vi "RFH-verify-R140_conversion.vi"(5 "Conversion Folder":path, 7 "Excel File Folder":path, 8 "error in (no error)":errorcluster, 9 "Max Frequency (6G)":dbl=6000000000.0, 10 "Min Frequency  (0.3G)":dbl=300000000.0) -> (0 "error out":errorcluster, 2 "All Good?":bool)   [LabVIEW 2020, in "RFH-Reflection_File_Handler.lvlib"]
doc: "Verifies converted R140 files against their Excel source files, value by value and in the min and max frequency range. Returns whether all are good."
uses:
  RFH-Reflection_File_Handler.lvlib
  RFH-common_data_format_element.ctl
panel:
  out "Range Good?":bool
  out "Values Good?":bool
  out "All Files in Dir":path[](array[path])
  out "value 4":T1
  out "value 3":T1
  out "value 2":T1
  out "value":T1
  out "Array":bool[](array[boolean])
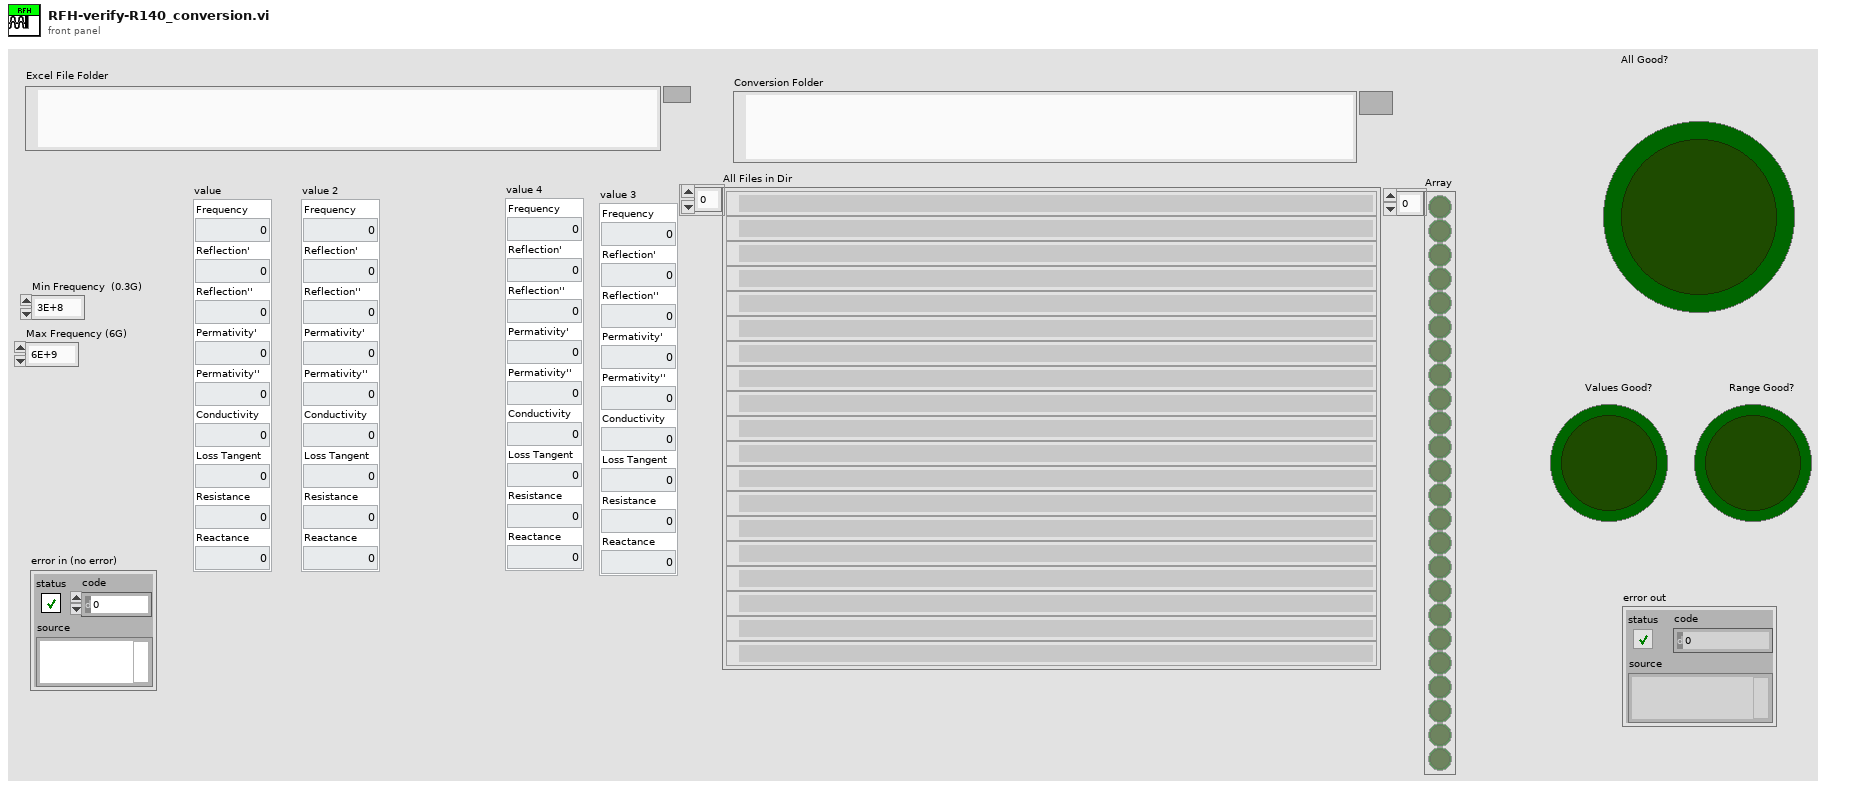
[diagram p1: front panel]
types:
  T1 = typedef "RFH-Reflection_File_Handler.lvlib/RFH-common_data_format_element.ctl" = cluster{"Frequency":dbl, "Reflection'":dbl, "Reflection''":dbl, "Permativity'":dbl, "Permativity''":dbl, "Conductivity":dbl, "Loss Tangent":dbl, "Resistance":dbl, "Reactance":dbl}
  T2 = typedef "RFH-Reflection_File_Handler.lvlib/RFH-common_data_format.ctl" = cluster{"Frequency":dbl[], "Reflection'":dbl[], "Reflection''":dbl[], "Permativity'":dbl[], "Permativity''":dbl[], "Conductivity":dbl[], "Loss Tangent":dbl[], "Resistance":dbl[], "Reactance":dbl[]}
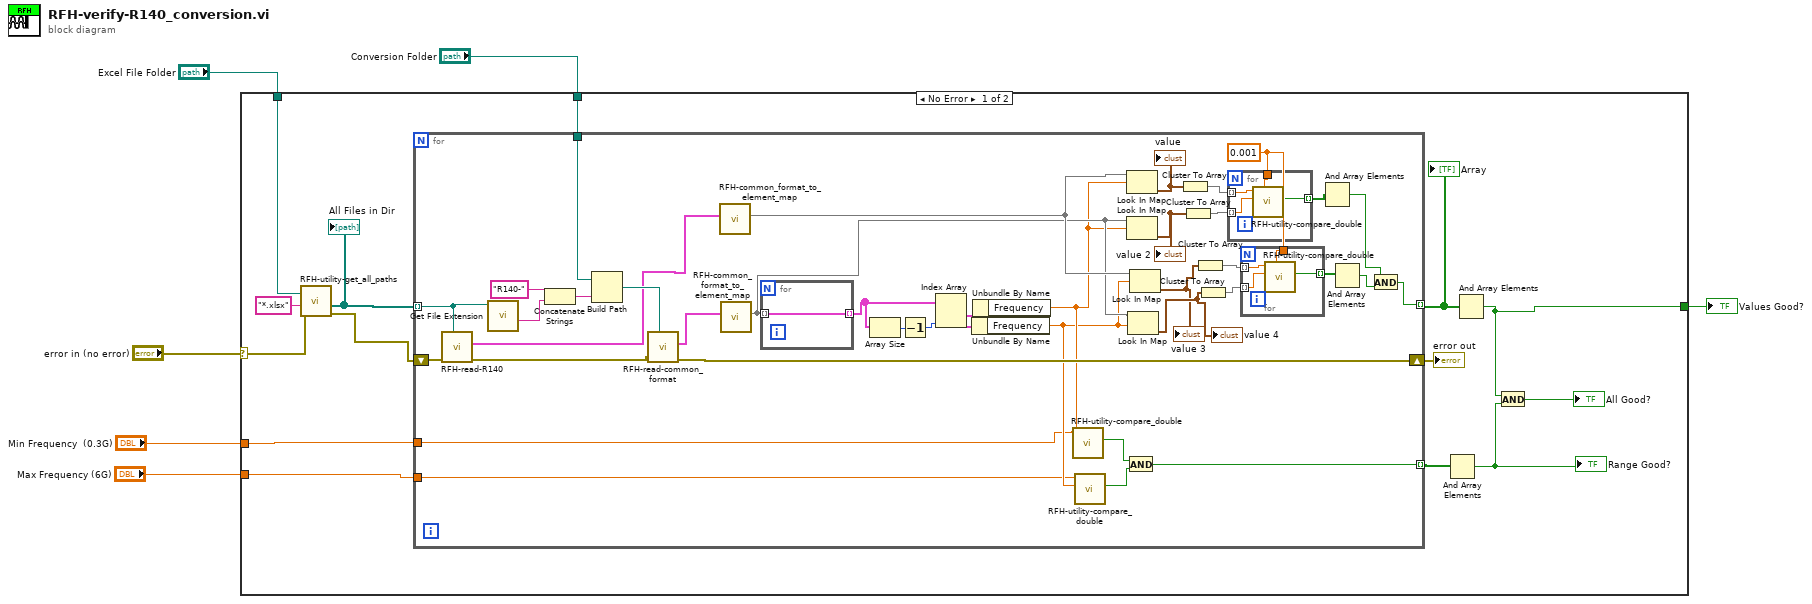
[diagram p0: block diagram]
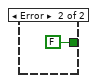
[diagram p2: hidden frame]
diagram:
  n1 = case shown="No Error" "error in (no error)" {
    selector: "error in (no error)" -> [w7 _]
    tunnel: "Excel File Folder" -> [w16 _]
    tunnel: "Conversion Folder" -> [w15 _]
    tunnel: "Min Frequency  (0.3G)" -> [w13 _]
    tunnel: "Max Frequency (6G)" -> [w12 _]
    tunnel: [w8 FALSE] -> w2
    frame No Error {
      n2 = call "RFH-utility-get_all_paths.vi"("Folder Path"=w16, "error in (no error)"=w7, "pattern"="*.xlsx") -> ("error out"=w19:errorcluster, "All Files in Dir"=w20:path[])  [unwired: 5 in, 2 out]
      "All Files in Dir" <- w20
      n3 = for {
        tunnel: w20 -> [w59] mode=indexing
        tunnel: w15 -> [w56]
        shift-right: [w51] -> w18
        shift-left: w19 -> [w54]
        tunnel: [w41] -> w14 mode=indexing
        tunnel: w13 -> [w23]
        tunnel: w12 -> [w22]
        tunnel: [w21] -> w10 mode=indexing
        w28 = 0.001 ("% tolerance (0.1)")
        n4 = call "RFH-read-R140.vi"("file path (dialog if empty)"=w59, "error in (no error)"=w54) -> ("error out"=w52:errorcluster, "Common Format"=w50:T2)  [unwired: 7 in, 1 out]
        n5 = call <vilib>:"Get File Extension.vi"("file"=w59) -> ("filename without extension"=w58:string)  [unwired: 6 in, 4 out]
        n6 = Concatenate Strings("R140-" ("string"), w58) -> (w57:string)
        n7 = Build Path(base path=w56, name or relative path=w57) -> (appended path=w53:path)
        n8 = call "RFH-read-common_format.vi"("file path (dialog if empty)"=w53, "error in"=w52) -> ("error out"=w51:errorcluster, "Common Format"=w49:T2)  [unwired: 8 in]
        n9 = call "RFH-common_format_to_element_map.vi"("Common Format"=w50) -> ("Element map"=w43:map{dbl, T1})  [unwired: 10 in]
        n10 = call "RFH-common_format_to_element_map.vi"("Common Format"=w49) -> ("Element map"=w42:map{dbl, T1})  [unwired: 10 in]
        n11 = for {
          tunnel: w42 -> [w68] mode=indexing
          tunnel: [w68] -> w46 mode=indexing
        }
        n12 = Array Size(array=w46) -> (size(s)=w47:i32)
        n13 = Decrement(x=w47) -> (x-1=w48:i32)
        n14 = Index Array(array=w46, index #2=w48) -> (element #1=w44:cluster{"Frequency":dbl, "Common Format":T1}, element #2=w45:cluster{"Frequency":dbl, "Common Format":T1})  [unwired: 1 in]
        n15 = Unbundle By Name(w45) -> ("Frequency"=w24:dbl)
        n16 = Unbundle By Name(w44) -> ("Frequency"=w25:dbl)
        n17 = call "RFH-utility-compare_double.vi"("New"=w25, "original"=w23) -> ("In Range?"=w26:bool)  [unwired: 9 in]
        n18 = call "RFH-utility-compare_double.vi"("New"=w24, "original"=w22) -> ("In Range?"=w27:bool)  [unwired: 9 in]
        n19 = And(x=w26, y=w27) -> (x .and. y?=w21:bool)
        n20 = Look In Map(map=w43, key=w25) -> (value=w40:T1)  [unwired: 1 in, 1 out]
        "value" <- w40
        n21 = Look In Map(map=w42, key=w25) -> (value=w39:T1)  [unwired: 1 in, 1 out]
        "value 2" <- w39
        n22 = Look In Map(map=w42, key=w24) -> (value=w34:T1)  [unwired: 1 in, 1 out]
        "value 4" <- w34
        n23 = Look In Map(map=w43, key=w24) -> (value=w33:T1)  [unwired: 1 in, 1 out]
        "value 3" <- w33
        n24 = Cluster To Array(cluster=w40) -> (array=w38:dbl[])
        n25 = Cluster To Array(cluster=w39) -> (array=w37:dbl[])
        n26 = Cluster To Array(cluster=w33) -> (array=w35:dbl[])
        n27 = Cluster To Array(cluster=w34) -> (array=w36:dbl[])
        n28 = for {
          tunnel: w38 -> [w67] mode=indexing
          tunnel: w37 -> [w66] mode=indexing
          tunnel: [w65] -> w29 mode=indexing
          tunnel: w28 -> [w64]
          n29 = call "RFH-utility-compare_double.vi"("% tolerance (0.1)"=w64, "New"=w66, "original"=w67) -> ("In Range?"=w65:bool)  [unwired: 8 in]
        }
        n30 = for {
          tunnel: w35 -> [w63] mode=indexing
          tunnel: w36 -> [w62] mode=indexing
          tunnel: [w61] -> w31 mode=indexing
          tunnel: w28 -> [w60]
          n31 = call "RFH-utility-compare_double.vi"("% tolerance (0.1)"=w60, "New"=w62, "original"=w63) -> ("In Range?"=w61:bool)  [unwired: 8 in]
        }
        n32 = And Array Elements(Boolean array=w29) -> (logical AND=w30:bool)
        n33 = And Array Elements(Boolean array=w31) -> (logical AND=w32:bool)
        n34 = And(x=w30, y=w32) -> (x .and. y?=w41:bool)
      }
      "error out" <- w18
      "Array" <- w14
      n35 = And Array Elements(Boolean array=w10) -> (logical AND=w9:bool)
      "Range Good?" <- w9
      n36 = And Array Elements(Boolean array=w14) -> (logical AND=w8:bool)
      n37 = And(x=w8, y=w9) -> (x .and. y?=→"All Good?":bool)
    }
    frame Error {
    }
  }
  "Values Good?" <- w2
